vi "Check.vi"(9 "log line":string, 10 "current file":refnum<file>, 11 "RolloverTrigger.Multi in":refnum<class "RolloverTrigger.Multi.lvclass">) -> (2 "rollover?":bool, 3 "RolloverTrigger.Multi out":refnum<class "RolloverTrigger.Multi.lvclass">)   [LabVIEW 2018, in "GLog.lvlib" / "RolloverTrigger.Multi.lvclass"]
doc: "Checks if the configured rollover condition has been met."
uses:
  RolloverTrigger.Multi.lvclass
  RolloverTrigger.Multi.lvclass/RolloverTrigger.Multi.ctl
  RolloverTrigger/RolloverTrigger.lvclass
panel:
  # "Connector Pane"
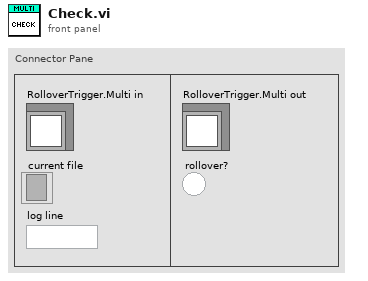
[diagram p1: front panel]
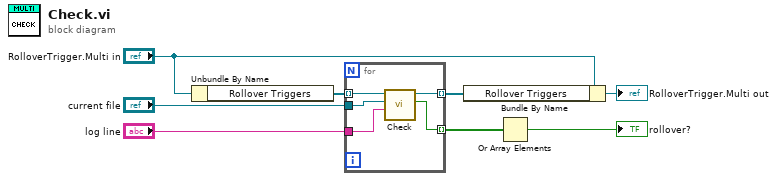
[diagram p0: block diagram]
diagram:
  n1 = Unbundle By Name("RolloverTrigger.Multi in") -> ("Rollover Triggers"=w8:refnum<class "RolloverTrigger.lvclass">[])
  n2 = for {
    tunnel: w8 -> [w13] mode=indexing
    tunnel: [w12] -> w5 mode=indexing
    tunnel: "current file" -> [w11]
    tunnel: "log line" -> [w10]
    tunnel: [w9] -> w2 mode=indexing
    n3 = call-dynamic "Check.vi"("log line"=w10, "current file"=w11, "RolloverTrigger in"=w13) -> ("rollover?"=w9:bool, "RolloverTrigger out"=w12:refnum<class "RolloverTrigger.lvclass">)  [unwired: 7 in]
  }
  n4 = Bundle By Name(cluster="RolloverTrigger.Multi in", "Rollover Triggers"=w5) -> (→"RolloverTrigger.Multi out":refnum<class "RolloverTrigger.Multi.lvclass">)
  n5 = Or Array Elements(Boolean array=w2) -> (logical OR=→"rollover?":bool)
